vi "test_LoadCommandlineArgs_AddPackedLibWithPathCheckDefaults.vi"() -> (3 "Pass?":bool)   [LabVIEW 2019, in "Tests.SolutionBuilder.lvlib"]
uses:
  Tests.SolutionBuilder.lvlib
  SolutionBuilder/Community/Options.ctl
  SolutionBuilder/ProjectItem/ProjectItem.lvclass/ProjectItem.ctl
  SolutionBuilder/SolutionBuilder.lvclass
  SolutionBuilder/ProjectItem/ProjectItem.lvclass
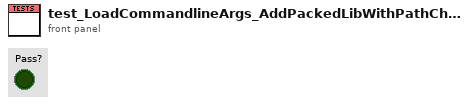
[diagram p1: front panel]
types:
  T1 = typedef "SolutionBuilder.lvlib/SolutionBuilder.lvclass/Options.ctl" = cluster{"Path":path, "Preview?":bool, "Quiet?":bool, "Log file":path, "Success file":path, "Rebuild?":bool, "Keep split projects?":bool, "Version string":string}
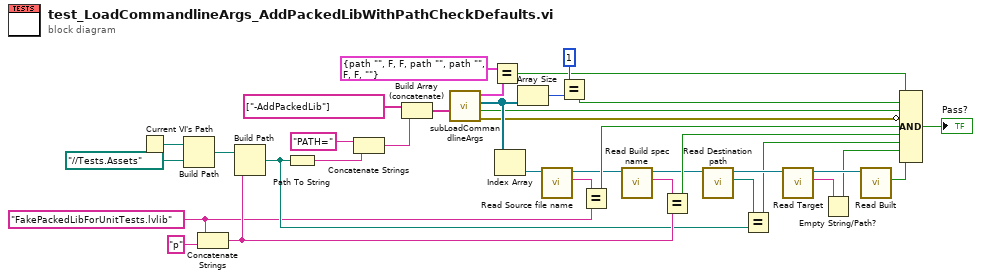
[diagram p0: block diagram]
diagram:
  w24 = "FakePackedLibForUnitTests.lvlib"
  n1 = Current VI's Path() -> (path=w13:path)
  n2 = Build Path(base path=w13, name or relative path=path "../../Tests.Assets" ("Path")) -> (appended path=w16:path)
  n3 = Concatenate Strings(w24, "p" ("string")) -> (w31:string)
  n4 = Build Path(base path=w16, name or relative path=w31) -> (appended path=w25:path)
  n5 = Path To String(path=w25) -> (string=w33:string)
  n6 = Concatenate Strings("PATH=" ("string"), w33) -> (w34:string)
  n7 = Build Array (concatenate)(string[] ["-AddPackedLib"] ("App.Args"), w34) -> (w14:string[])
  n8 = call "subLoadCommandlineArgs.vi"("App.Args"=w14) -> ("error out"=w7:errorcluster, "From command line?"=w3:bool, "Pre-built libraries"=w15:refnum<class "ProjectItem.lvclass">[], "Options"=w5:T1)  [unwired: 5 in, 2 out]
  n9 = Equal?(x=T1 {"Path"=path "", "Preview?"=FALSE, "Quiet?"=FALSE, "Log file"=path "", "Success file"=path "", "Rebuild?"=FALSE, "Keep split projects?"=FALSE, "Version string"=""} ("Options"), y=w5) -> (x = y?=w4:bool)
  n10 = Index Array(array=w15) -> (element=w17:refnum<class "ProjectItem.lvclass">)  [unwired: 1 in]
  n11 = Array Size(array=w15) -> (size(s)=w8:i32)
  n12 = call "Read Source file name.vi"("ProjectItem in"=w17) -> ("Source file name"=w22:string, "ProjectItem out"=w19:refnum<class "ProjectItem.lvclass">)  [unwired: 9 in]
  n13 = Equal?(x=1, y=w8) -> (x = y?=w10:bool)
  n14 = Equal?(x=w22, y=w24) -> (x = y?=w27:bool)
  n15 = call "Read Build spec name.vi"("ProjectItem in"=w19) -> ("Build spec name"=w23:string, "ProjectItem out"=w20:refnum<class "ProjectItem.lvclass">)  [unwired: 9 in]
  n16 = Equal?(x=w23, y=w31) -> (x = y?=w28:bool)
  n17 = call "Read Destination path.vi"("ProjectItem in"=w20) -> ("Destination path"=w26:path, "ProjectItem out"=w35:refnum<class "ProjectItem.lvclass">)  [unwired: 9 in]
  n18 = Equal?(x=w26, y=w25) -> (x = y?=w29:bool)
  n19 = call "Read Target.vi"("ProjectItem in"=w35) -> ("Target"=w2:string, "ProjectItem out"=w36:refnum<class "ProjectItem.lvclass">)  [unwired: 9 in]
  n20 = Empty String/Path?(string/path=w2) -> (empty?=w1:bool)
  n21 = call "Read Built.vi"("ProjectItem in"=w36) -> ("Built"=w21:bool)  [unwired: 9 in, 1 out]
  n22 = Compound Arithmetic op=AND(w4, w10, w3, invert w7, w27, w28, w29, w1, w21) -> (→"Pass?":bool)
